vi "MoveLayers.vi"(8 "error in":errorcluster, 10 "Arrow Up":bool, 11 "Data in":T1={"Class"={"Ants"=refnum, "Layer"=refnum, "Templates"=refnum, "Icon"=refnum, "Glyph"=refnum, "Settings"=refnum, "Tools"=refnum, "History"=refnum}, "Ref"={"Add Layer"=refnum, "Remove Layer"=refnum, "Line Text"=[], "Body Text Spec"=refnum, "DNL_Font"=refnum, "glyph path str"=refnum, "templates path str"=refnum, "Arrow Up"=refnum, "Arrow Down"=refnum, "IE VI Ref"=refnum, "Glyphs tree"=refnum, "Templates tree"=refnum, "Layer Icon Text"=refnum, "Layer Template"=refnum, "Body Text"=refnum, "Search Templates"=refnum, "TextMarker"=refnum, "Tab Control"=refnum, "Search Glyphs"=refnum, "Line Color"=refnum, "DNL_Glyphs []"=refnum, "Fill Color"=refnum, "Tools"=refnum, "Icon"=refnum, "Preview"=refnum, "Ants"=refnum, "Terminals"=refnum, "menu reference"=refnum, "LayerNames"=[], "GlyphLoadAnimation"=refnum, "TemplateLoadAnimation"=refnum, "refreshGlyphs"=refnum, "refreshTemplates"=refnum}, "Support"={"AntsRect"={"left"=0, "top"=0, "right"=0, "bottom"=0}, "Mouse Move Coords"={"Horizontal"=0, "Vertical"=0}, "Mouse Down Coords"={"Horizontal"=0, "Vertical"=0}, "Temp Coord"={"Horizontal"=0, "Vertical"=0}, "Action"=enum."Default", "Edge Color"=4914962, "Fill Color"=16860, "Mouse Down?"=FALSE, "Draft Mode?"=FALSE, "Temp Icon"=bytes[3102], "CTRL Pressed"=FALSE, "Move Selection?"=FALSE, "AntsRect Orig"={"left"=0, "top"=0, "right"=0, "bottom"=0}, "Text"="", "TM Set?"=FALSE, "Mouse inside icon?"=FALSE, "Tool (old value)"=0, "Pencil Move Color"=0, "Swap Colors?"=FALSE, "Shift pressed?"=FALSE}}) -> (0 "error out":errorcluster, 3 "Data out":T1={"Class"={"Ants"=refnum, "Layer"=refnum, "Templates"=refnum, "Icon"=refnum, "Glyph"=refnum, "Settings"=refnum, "Tools"=refnum, "History"=refnum}, "Ref"={"Add Layer"=refnum, "Remove Layer"=refnum, "Line Text"=[], "Body Text Spec"=refnum, "DNL_Font"=refnum, "glyph path str"=refnum, "templates path str"=refnum, "Arrow Up"=refnum, "Arrow Down"=refnum, "IE VI Ref"=refnum, "Glyphs tree"=refnum, "Templates tree"=refnum, "Layer Icon Text"=refnum, "Layer Template"=refnum, "Body Text"=refnum, "Search Templates"=refnum, "TextMarker"=refnum, "Tab Control"=refnum, "Search Glyphs"=refnum, "Line Color"=refnum, "DNL_Glyphs []"=refnum, "Fill Color"=refnum, "Tools"=refnum, "Icon"=refnum, "Preview"=refnum, "Ants"=refnum, "Terminals"=refnum, "menu reference"=refnum, "LayerNames"=[], "GlyphLoadAnimation"=refnum, "TemplateLoadAnimation"=refnum, "refreshGlyphs"=refnum, "refreshTemplates"=refnum}, "Support"={"AntsRect"={"left"=0, "top"=0, "right"=0, "bottom"=0}, "Mouse Move Coords"={"Horizontal"=0, "Vertical"=0}, "Mouse Down Coords"={"Horizontal"=0, "Vertical"=0}, "Temp Coord"={"Horizontal"=0, "Vertical"=0}, "Action"=enum."Default", "Edge Color"=4914962, "Fill Color"=16860, "Mouse Down?"=FALSE, "Draft Mode?"=FALSE, "Temp Icon"=bytes[3102], "CTRL Pressed"=FALSE, "Move Selection?"=FALSE, "AntsRect Orig"={"left"=0, "top"=0, "right"=0, "bottom"=0}, "Text"="", "TM Set?"=FALSE, "Mouse inside icon?"=FALSE, "Tool (old value)"=0, "Pencil Move Color"=0, "Swap Colors?"=FALSE, "Shift pressed?"=FALSE}})   [LabVIEW 2020]
uses:
  Class/Ants/Ants.lvclass
  Class/FakedArray/FakedArray.lvclass
  vi.lib/LabVIEW Icon API/lv_icon/Classes/Icon/Icon.lvclass
  Class/Icon Library/Glyph.lvclass
  Class/Settings/Settings.lvclass
  Class/Tools/Tools Paint.lvclass
  History/History/History.lvclass
  History/History.lvlib
  <vilib>/Utility/miscctls.llb/LVPoint32TypeDef.ctl
  Controls/SupportClass_Action.ctl
  vi.lib/LabVIEW Icon API/lv_icon/Controls/IEColor.ctl
  Controls/Support Cluster.ctl
  lv_icon.lvlib
  Controls/References Cluster.ctl
  Controls/IE Classes.ctl
  Controls/Global Data.ctl
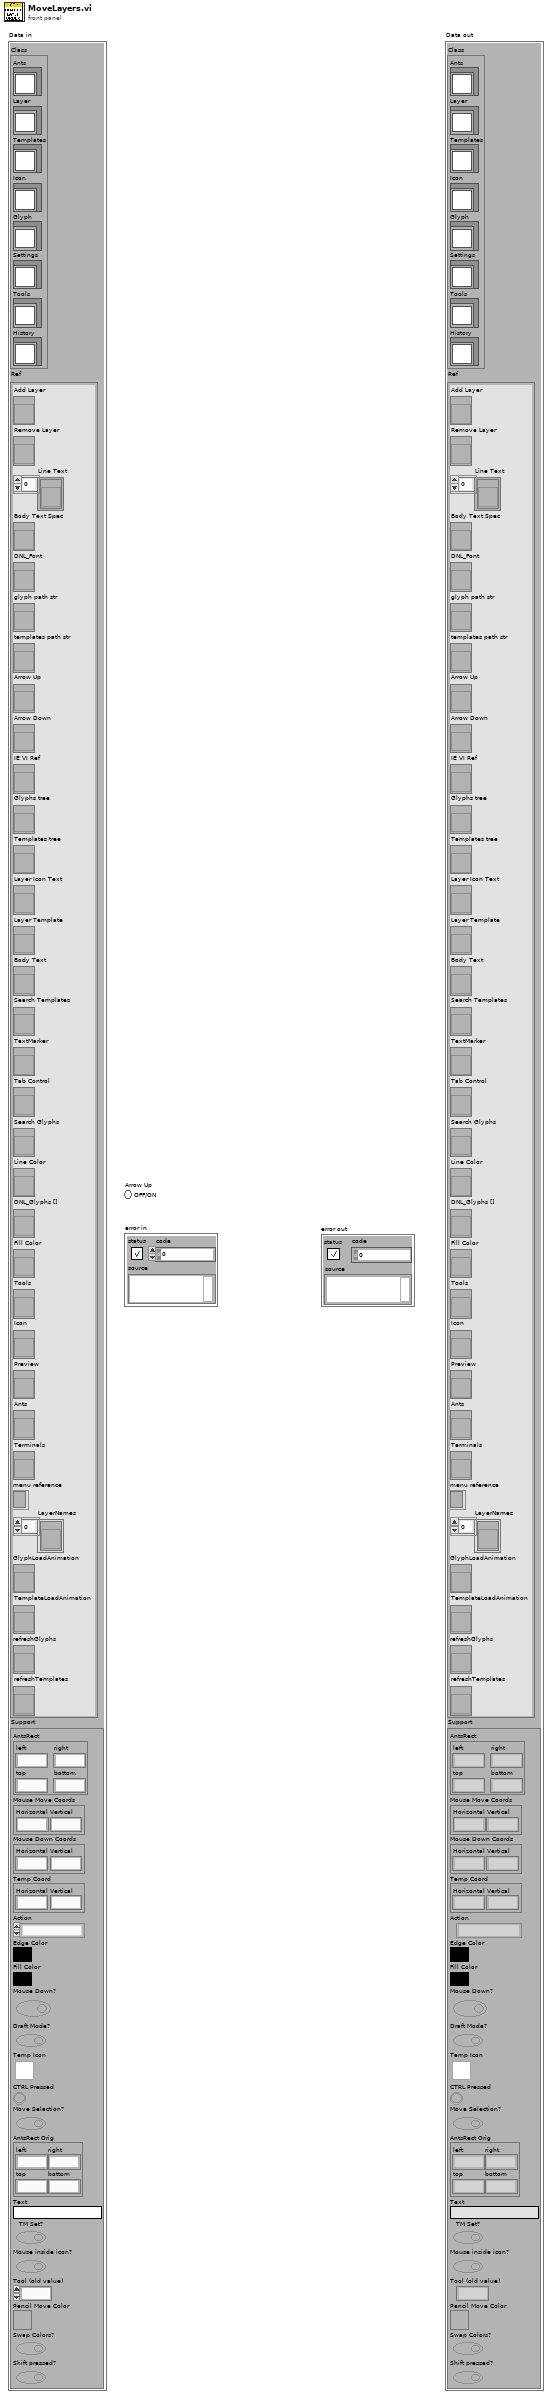
[diagram p1: front panel]
types:
  T1 = typedef "lv_icon.lvlib/Global Data.ctl" = cluster{"Class":T2, "Ref":T3, "Support":T4}
  T2 = typedef "lv_icon.lvlib/IE Classes.ctl" = cluster{"Ants":refnum<class "Ants.lvclass">, "Layer":refnum<class "FakedArray.lvclass">, "Templates":refnum<class "FakedArray.lvclass">, "Icon":refnum<class "Icon.lvclass">, "Glyph":refnum<class "Glyph.lvclass">, "Settings":refnum<class "Settings.lvclass">, "Tools":refnum<class "Tools Paint.lvclass">, "History":refnum<class "History.lvclass">}
  T3 = typedef "lv_icon.lvlib/References Cluster.ctl" = cluster{"Add Layer":refnum<vi>, "Remove Layer":refnum<vi>, "Line Text":refnum<vi>[], "Body Text Spec":refnum<vi>, "DNL_Font":refnum<vi>, "glyph path str":refnum<vi>, "templates path str":refnum<vi>, "Arrow Up":refnum<vi>, "Arrow Down":refnum<vi>, "IE VI Ref":refnum<vi>, "Glyphs tree":refnum<vi>, "Templates tree":refnum<vi>, "Layer Icon Text":refnum<vi>, "Layer Template":refnum<vi>, "Body Text":refnum<vi>, "Search Templates":refnum<vi>, "TextMarker":refnum<vi>, "Tab Control":refnum<vi>, "Search Glyphs":refnum<vi>, "Line Color":refnum<vi>, "DNL_Glyphs []":refnum<vi>, "Fill Color":refnum<vi>, "Tools":refnum<vi>, "Icon":refnum<vi>, "Preview":refnum<vi>, "Ants":refnum<vi>, "Terminals":refnum<vi>, "menu reference":refnum<k9>, "LayerNames":refnum<vi>[], "GlyphLoadAnimation":refnum<vi>, "TemplateLoadAnimation":refnum<vi>, "refreshGlyphs":refnum<vi>, "refreshTemplates":refnum<vi>}
  T4 = typedef "lv_icon.lvlib/Support Cluster.ctl" = cluster{"AntsRect":cluster{"left":i16, "top":i16, "right":i16, "bottom":i16}, "Mouse Move Coords":T5, "Mouse Down Coords":T5, "Temp Coord":T5, "Action":T6, "Edge Color":T7, "Fill Color":T7, "Mouse Down?":bool, "Draft Mode?":bool, "Temp Icon":picture, "CTRL Pressed":bool, "Move Selection?":bool, "AntsRect Orig":cluster{"left":i16, "top":i16, "right":i16, "bottom":i16}, "Text":string, "TM Set?":bool, "Mouse inside icon?":bool, "Tool (old value)":u32, "Pencil Move Color":u32, "Swap Colors?":bool, "Shift pressed?":bool}
  T5 = typedef "LVPoint32TypeDef.ctl" = cluster{"Horizontal":i32, "Vertical":i32}
  T6 = typedef "SupportClass_Action.ctl" = enum16{"Default", "Move Selection", "Glyph Library", "Tool"}
  T7 = typedef "IEColor.ctl" = u32
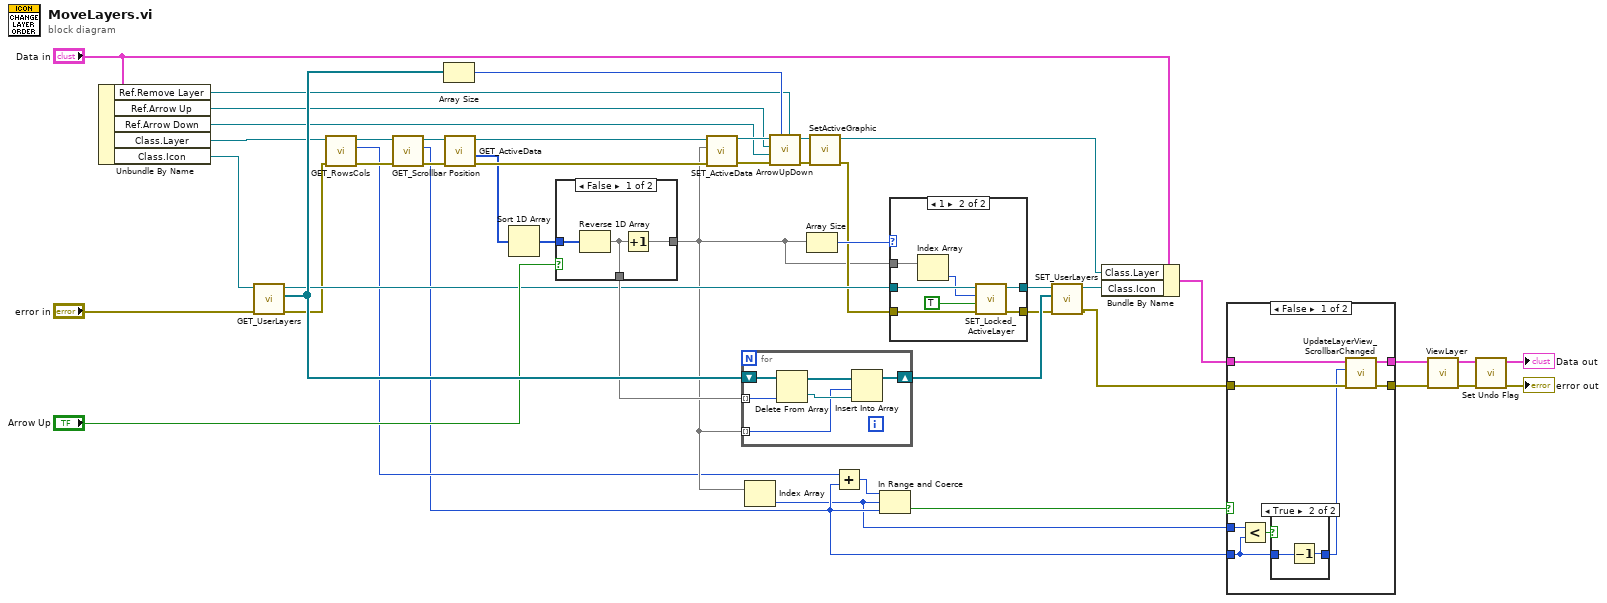
[diagram p0: block diagram]
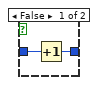
[diagram p2: hidden frame]
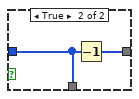
[diagram p5: hidden frame]
diagram:
  n1 = Unbundle By Name("Data in") -> ("Ref.Remove Layer"=w4:refnum<vi>, "Ref.Arrow Up"=w23:refnum<vi>, "Ref.Arrow Down"=w24:refnum<vi>, "Class.Layer"=w9:refnum<class "FakedArray.lvclass">, "Class.Icon"=w27:refnum<class "Icon.lvclass">)
  n2 = call-dynamic "GET_UserLayers.vi"("error in (no error)"="error in", "Icon.lvclass in"=w27) -> ("error out"=w12:errorcluster, "All Layers"=w40:refnum<class "Layer.lvclass">[], "Icon.lvclass out"=w29:refnum<class "Icon.lvclass">)  [unwired: 7 out]
  n3 = call-dynamic "GET_RowsCols.vi"("error in (no error)"=w12, "FakedArray.lvclass in"=w9) -> ("error out"=w11:errorcluster, "# Rows"=w8:i32, "FakedArray.lvclass out"=w10:refnum<class "FakedArray.lvclass">)  [unwired: 7 out]
  n4 = call-dynamic "GET_Scrollbar Position.vi"("error in (no error)"=w11, "FakedArray.lvclass in"=w10) -> ("error out"=w13:errorcluster, "Scrollbar Position"=w6:i32, "FakedArray.lvclass out"=w14:refnum<class "FakedArray.lvclass">)  [unwired: 7 out]
  n5 = Array Size(array=w40) -> (size(s)=w39:i32)
  n6 = call-dynamic "GET_ActiveData.vi"("error in (no error)"=w13, "FakedArray in"=w14) -> ("error out"=w46:errorcluster, "Active Data []"=w36:i32[], "FakedArray out"=w42:refnum<class "FakedArray.lvclass">)  [unwired: 7 out]
  n7 = Sort 1D Array(array=w36) -> (sorted array=w34:i32[])
  n8 = case shown="False" "Arrow Up" {
    tunnel: w34 -> [w49 w50]
    tunnel: [w48 w51] -> w15
    tunnel: [w47 w50] -> w33
    frame False {
      n9 = Reverse 1D Array(array=w49) -> (reversed array=w47:i32[])
      n10 = Increment(x=w47) -> (x+1=w48:i32[])
    }
    frame True {
      n11 = Decrement(x=w50) -> (x-1=w51:i32[])
    }
  }
  n12 = call-dynamic "SET_ActiveData.vi"("error in (no error)"=w46, "Active Data"=w15, "FakedArray.lvclass in"=w42) -> ("error out"=w43:errorcluster, "FakedArray.lvclass out"=w41:refnum<class "FakedArray.lvclass">)  [unwired: 7 out]
  n13 = for {
    shift-right: [w54] -> w45
    shift-left: w40 -> [w57]
    tunnel: w33 -> [w56] mode=indexing
    tunnel: w15 -> [w52] mode=indexing
    n14 = Delete From Array(array=w57, index=w56) -> (deleted portion=w53:refnum<class "Layer.lvclass">, array with subset deleted=w55:refnum<class "Layer.lvclass">[])  [unwired: 1 in]
    n15 = Insert Into Array(array=w55, index=w52, new element=w53) -> (w54:refnum<class "Layer.lvclass">[])
  }
  n16 = Index Array(array=w15) -> (element=w5:i32)  [unwired: 1 in]
  n17 = call "ArrowUpDown.vi"("Remove Layer"=w4, "# Layers"=w39, "error in (no error)"=w43, "Arrow Down"=w24, "Arrow Up"=w23, "FakedArray in"=w41) -> ("error out"=w37:errorcluster, "FakedArray out"=w38:refnum<class "FakedArray.lvclass">)  [unwired: 4 out]
  n18 = Array Size(array=w15) -> (size(s)=w30:i32)
  n19 = call-dynamic "SetActiveGraphic.vi"("error in (no error)"=w37, "FakedArray in"=w38) -> ("error out"=w28:errorcluster, "FakedArray out"=w22:refnum<class "FakedArray.lvclass">)  [unwired: 4 in, 4 out]
  n20 = Add(x=w8, y=w6) -> (x+y=w16:i32)
  n21 = In Range and Coerce(upper limit=w16, x=w5, lower limit=w6) -> (In Range?=w7:bool)  [unwired: 1 out]
  n22 = case shown="1" w30 {
    tunnel: [w59 w66] -> w32
    tunnel: [w58 w65] -> w31
    tunnel: w29 -> [w59 w64]
    tunnel: w28 -> [w58 w63]
    tunnel: w15 -> [_ w62]
    frame 0, Default {
    }
    frame 1 {
      n23 = Index Array(array=w62) -> (element=w61:i32)  [unwired: 1 in]
      n24 = call-dynamic "SET_Locked_ActiveLayer.vi"("error in (no error)"=w63, "Layers Locked?"=TRUE, "Active Layer"=w61, "Icon.lvclass in"=w64) -> ("error out"=w65:errorcluster, "Icon.lvclass out"=w66:refnum<class "Icon.lvclass">)  [unwired: 6 out]
    }
  }
  n25 = call-dynamic "SET_UserLayers.vi"("error in (no error)"=w31, "Layers"=w45, "Icon.lvclass in"=w32) -> ("error out"=w18:errorcluster, "Icon.lvclass out"=w25:refnum<class "Icon.lvclass">)  [unwired: 7 in]
  n26 = Bundle By Name(cluster="Data in", "Class.Layer"=w22, "Class.Icon"=w25) -> (w19:T1)
  n27 = case shown="False" w7 {
    tunnel: [w74 w80] -> w20
    tunnel: w19 -> [w73 w80]
    tunnel: w18 -> [w72 w79]
    tunnel: [w71 w79] -> w17
    tunnel: w6 -> [w67 _]
    tunnel: w5 -> [w68 _]
    frame False {
      n28 = Less?(x=w68, y=w67) -> (x < y?=w70:bool)
      n29 = case shown="True" w70 {
        tunnel: w67 -> [w76 w78]
        tunnel: [w75 w77] -> w69
        frame False {
          n30 = Increment(x=w76) -> (x+1=w75:i32)
        }
        frame True {
          n31 = Decrement(x=w78) -> (x-1=w77:i32)
        }
      }
      n32 = call "UpdateLayerView_ScrollbarChanged.vi"("error in"=w72, "Scrollbar Position"=w69, "Data in"=w73) -> ("error out"=w71:errorcluster, "Data out"=w74:T1)  [unwired: 7 out]
    }
    frame True {
    }
  }
  n33 = call "ViewLayer.vi"("error in (no error)"=w17, "Data in"=w20) -> ("error out"=w44:errorcluster, "Data out"=w2:T1)  [unwired: 3 in, 5 out]
  n34 = call "Set Undo Flag.vi"("error in"=w44, "Data in"=w2) -> ("error out"=→"error out":errorcluster, "Data out"=→"Data out":T1)  [unwired: 8 in]
